vi "RemoteVI Set Server Loop Inputs.vi"(0 "Server Loop":refnum<vi>, 1 "stop notifier name":string, 2 "share":T1, 5 "VI":refnum<vi>, 7 "port":u16=8088, 9 "fps":dbl=20.0, 11 "error in":errorcluster) -> (4 "Server Loop out":refnum<vi>, 15 "error out":errorcluster)   [LabVIEW 2020, in "RemoteVI.lvlib"]
doc: "Sets the controls VI, port, fps, stop notifier name and share of the Server Loop that Server Loop references (Set Control Value [Variant], one after the other) before RemoteVI Start.vi runs it. Nothing is set on an incoming error."
uses:
  RemoteVI.lvlib
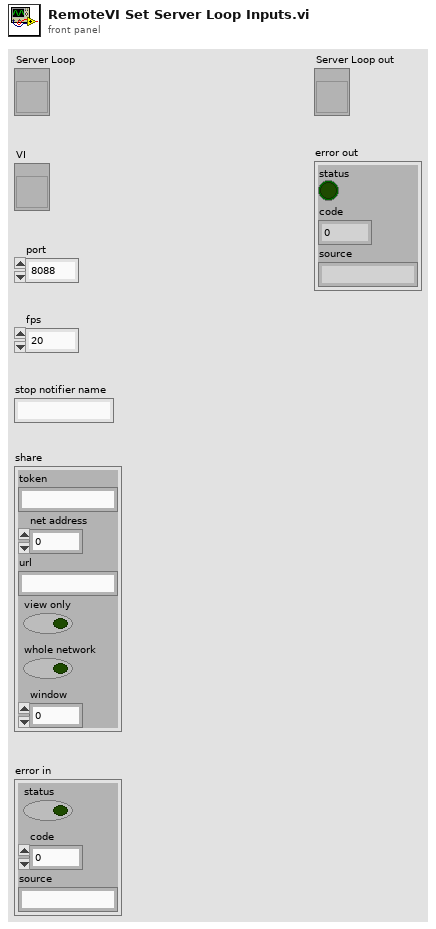
[diagram p1: front panel]
types:
  T1 = cluster{"token":string, "net address":u32, "url":string, "view only":bool, "whole network":bool, "window":u64}
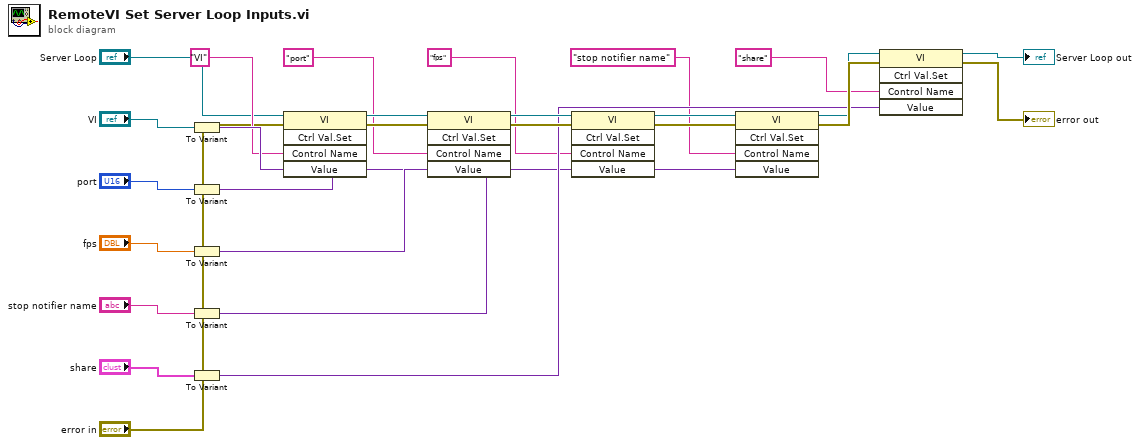
[diagram p0: block diagram]
diagram:
  n1 = To Variant(anything="VI") -> (Variant=w12:variant)
  n2 = To Variant(anything="port") -> (Variant=w13:variant)
  n3 = To Variant(anything="fps") -> (Variant=w14:variant)
  n4 = To Variant(anything="stop notifier name") -> (Variant=w15:variant)
  n5 = To Variant(anything="share") -> (Variant=w17:variant)
  n6 = invoke class="VI" method="Ctrl Val.Set"(reference="Server Loop", error in="error in", "Control Name"="VI", "Value"=w12) -> (reference out=w18:refnum<vi>, error out=w19:errorcluster)  [unwired: 1 in, 3 out]
  n7 = invoke class="VI" method="Ctrl Val.Set"(reference=w18, error in=w19, "Control Name"="port", "Value"=w13) -> (reference out=w20:refnum<vi>, error out=w21:errorcluster)  [unwired: 1 in, 3 out]
  n8 = invoke class="VI" method="Ctrl Val.Set"(reference=w20, error in=w21, "Control Name"="fps", "Value"=w14) -> (reference out=w22:refnum<vi>, error out=w23:errorcluster)  [unwired: 1 in, 3 out]
  n9 = invoke class="VI" method="Ctrl Val.Set"(reference=w22, error in=w23, "Control Name"="stop notifier name", "Value"=w15) -> (reference out=w24:refnum<vi>, error out=w25:errorcluster)  [unwired: 1 in, 3 out]
  n10 = invoke class="VI" method="Ctrl Val.Set"(reference=w24, error in=w25, "Control Name"="share", "Value"=w17) -> (reference out=→"Server Loop out":refnum<vi>, error out=→"error out":errorcluster)  [unwired: 1 in, 3 out]
